vi "DAC Save Results.vi"(8 "error in":errorcluster, 9 "Log Details?":bool, 10 "tdms file":refnum<k34>, 11 "DAC Inclino in":refnum<class "DAC Inclinometer.lvclass">) -> (0 "error out":errorcluster)   [LabVIEW 2019, in "DAC.lvlib" / "DAC Inclinometer.lvclass"]
uses:
  DAC Inclinometer.lvclass
  C:/Users/wg/Documents/LV_Projects/test-stand/App/DAC/DAC.lvclass
  DAC.lvclass/DAC.ctl
  DAC Inclinometer.lvclass/DAC Inclinometer.ctl
  DAC.lvclass
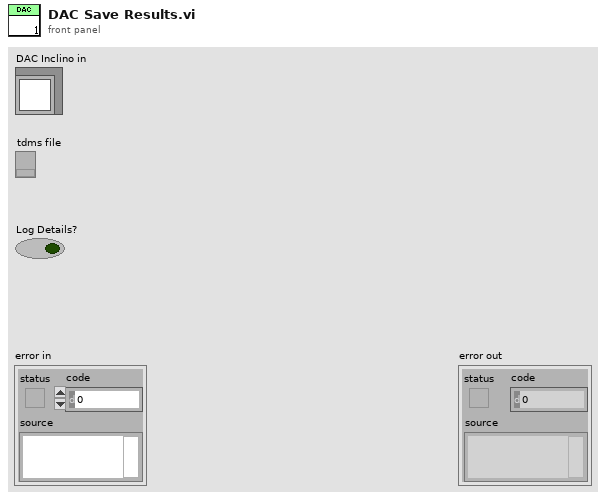
[diagram p1: front panel]
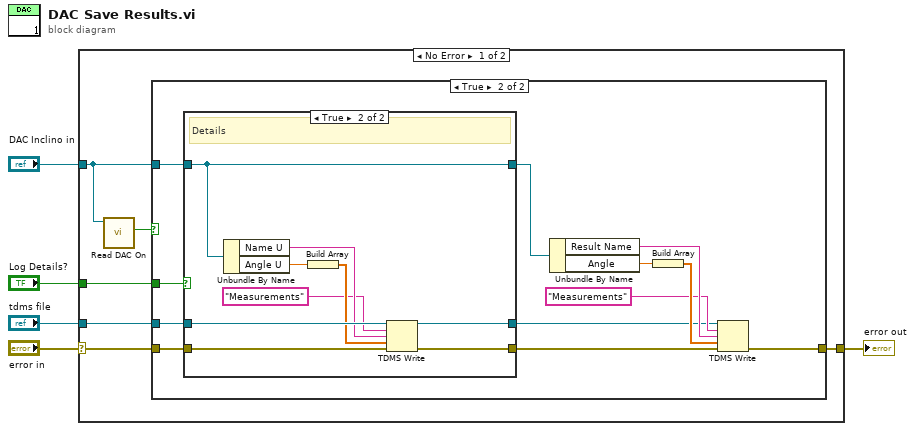
[diagram p0: block diagram]
diagram:
  n1 = case shown="No Error" "error in" {
    selector: "error in" -> [w8 w37]
    tunnel: "DAC Inclino in" -> [w11 _]
    tunnel: "tdms file" -> [w9 _]
    tunnel: [w7 w37] -> w3
    tunnel: "Log Details?" -> [w6 _]
    frame No Error {
      n2 = call "Read DAC On.vi"("DAC in"=w11) -> ("DAC On"=w10:bool)  [unwired: 8 in, 2 out]
      n3 = case shown="True" w10 {
        tunnel: w11 -> [_ w20]
        tunnel: w9 -> [_ w18]
        tunnel: w8 -> [w12 w17]
        tunnel: [w12 w13] -> w7
        tunnel: w6 -> [_ w19]
        frame False {
        }
        frame True {
          n4 = case shown="True" w19 {
            tunnel: w18 -> [w26 w36]
            tunnel: w17 -> [w27 w32]
            tunnel: w20 -> [w25 w31]
            tunnel: [w27 w29] -> w14
            tunnel: [w26 w30] -> w15
            tunnel: [w25 w31] -> w16
            frame False {
            }
            frame True {
              # "Details"
              n5 = Unbundle By Name(w31) -> ("Name U"=w33:string, "Angle U"=w35:dbl)
              n6 = Build Array(w35) -> (w34:dbl[])
              n7 = TDMS Write(0:w36, 5:"Measurements" ("group name in (Untitled)"), 7:w33, 9:w34, 11:w32) -> (4:w30:refnum<k34>, 15:w29:errorcluster)  [unwired: 1 in, 2 out]
            }
          }
          n8 = Unbundle By Name(w16) -> ("Result Name"=w22:string, "Angle"=w24:dbl)
          n9 = Build Array(w24) -> (w23:dbl[])
          n10 = TDMS Write(0:w15, 5:"Measurements" ("group name in (Untitled)"), 7:w22, 9:w23, 11:w14) -> (15:w13:errorcluster)  [unwired: 1 in, 3 out]
        }
      }
    }
    frame Error {
    }
  }
  "error out" <- w3
